vi "input.vi"(8 "error in":errorcluster, 10 "input allocation":T1, 11 "DAQmx Watchdog runtime in":refnum<class "DAQmx Watchdog runtime.lvclass">) -> (0 "error out":errorcluster, 2 "input data":T1, 3 "DAQmx Watchdog runtime out":refnum<class "DAQmx Watchdog runtime.lvclass">)   [LabVIEW 2014, in "DAQmx Watchdog runtime.lvclass"]
doc: "Provides an interface for reading data from a module at runtime. While this interface performs no operations, a child should provide an override which may read from any open sessions, references, or interfaces."
uses:
  DAQmx Watchdog runtime.lvclass
  <vilib>/NI/Tag Bus/table/data table.ctl
  input user data.ctl
  DAQmx Watchdog runtime.lvclass/DAQmx Watchdog runtime.ctl
  <vilib>/NI/Syslog Wrapper - Linux/write syslog.vi
  <vilib>/Utility/LVClass/Get LV Class Name.vi
  <resource>/objmgr/daqmx.rc
  <vilib>/NI/Tag Bus Module Framework/runtime/TBM module execution interface.lvclass
  <vilib>/NI/Tag Bus/table/data table.lvlib
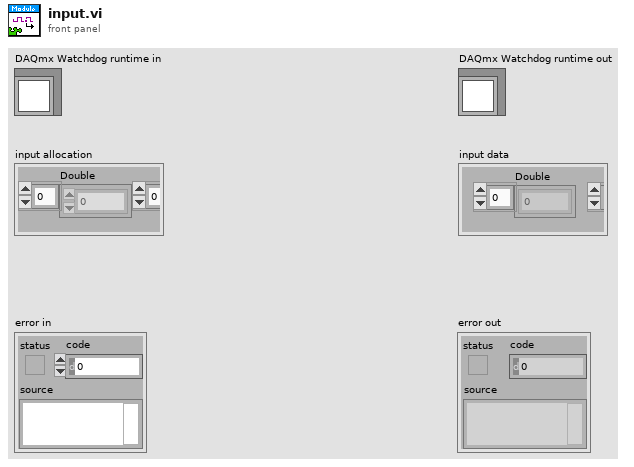
[diagram p1: front panel]
types:
  T1 = typedef "tag bus.lvlib/data table.lvlib/data table.ctl" = cluster{"Double":dbl[], "Single":sgl[], "I64":i64[], "I32":i32[], "I16":i16[], "I8":i8[], "U64":u64[], "U32":u32[], "U16":u16[], "U8":u8[], "Boolean":bool[], "String":string[], "Array of Double":cluster{"DBL Array":dbl[]}[], "Array of Single":cluster{"SGL Array":sgl[]}[], "Array of I64":cluster{"I64 Array":i64[]}[], "Array of I32":cluster{"I32 Array":i32[]}[], "Array of I16":cluster{"I16 Array":i16[]}[], "Array of I8":cluster{"I8 Array":i8[]}[], "Array of U64":cluster{"U64 Array":u64[]}[], "Array of U32":cluster{"U32 Array":u32[]}[], "Array of U16":cluster{"U16 Array":u16[]}[], "Array of U8":cluster{"U8 Array":u8[]}[], "Array of Boolean":cluster{"Boolean Array":bool[]}[], "Array of String":cluster{"String Array":string[]}[]}
  T2 = typedef "DAQmx Watchdog runtime.lvclass/input user data.ctl" = cluster{"Watchdog Expired":bool}
  T3 = typedef "DAQmx Watchdog configuration.lvclass/input data indices.ctl" = cluster{"Boolean.Watchdog Expired":i32}
  T4 = enum16{"Emergency", "Alert", "Critical", "Error", "Warning", "Notice", "Informational", "Debug"}
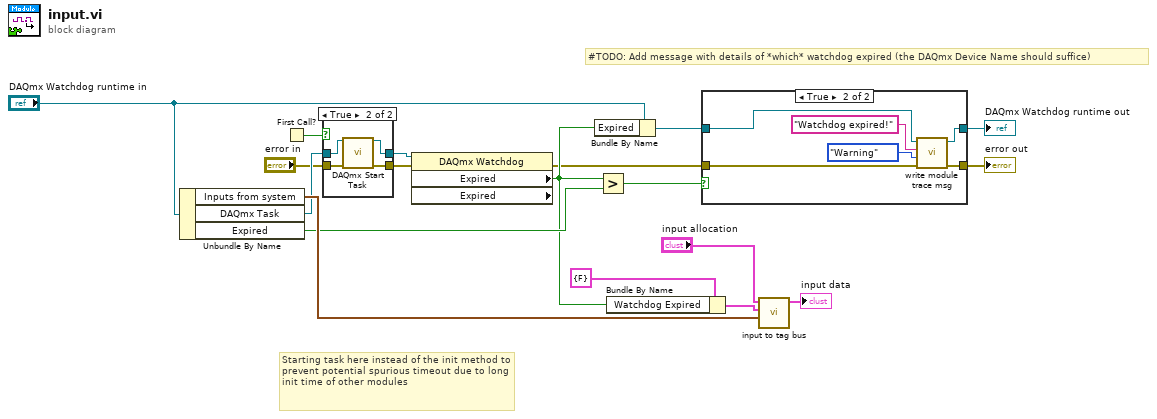
[diagram p0: block diagram]
diagram:
  # "#TODO: Add message with details of *which* watchdog expired (the DAQmx Device Name should suffice)"
  # "Starting task here instead of the init method to prevent potential spurious timeout due to long init time of other modules"
  n1 = Unbundle By Name("DAQmx Watchdog runtime in") -> ("Inputs from system"=w16:T3, "DAQmx Task"=w12:refnum<k21>, "Expired"=w8:bool)
  n2 = First Call?() -> (First Call?: T/F=w13:bool)
  n3 = case shown="True" w13 {
    tunnel: w12 -> [w19 w24]
    tunnel: "error in" -> [w20 w23]
    tunnel: [w20 w22] -> w10
    tunnel: [w19 w21] -> w9
    frame False {
    }
    frame True {
      n4 = call <vilib>:"DAQmx Start Task.vi"("task/channels in"=w24, "error in"=w23) -> ("task out"=w21:refnum<k21>, "error out"=w22:errorcluster)  [unwired: 12 in]
    }
  }
  n5 = property class="DAQmx Watchdog" props=["Expired", "Expired"](reference=w9, error in=w10) -> (error out=w4:errorcluster, "Expired"=w6:bool)  [unwired: 2 out]
  n6 = Bundle By Name(cluster="DAQmx Watchdog runtime in", "Expired"=w6) -> (w5:refnum<class "DAQmx Watchdog runtime.lvclass">)
  n7 = Greater?(x=w6, y=w8) -> (0:w1:bool)
  n8 = Bundle By Name(cluster=T2 {"Watchdog Expired"=FALSE} ("data cluster"), "Watchdog Expired"=w6) -> (w14:T2)
  n9 = case shown="True" w1 {
    tunnel: w5 -> [w25 w32]
    tunnel: w4 -> [w26 w31]
    tunnel: [w26 w30] -> w3
    tunnel: [w25 w27] -> w2
    frame False {
    }
    frame True {
      n10 = call <vilib>:"write module trace msg.vi"("error in (no error)"=w31, "Priority"=T4."Warning", "message"="Watchdog expired!", "module in"=w32) -> ("error out"=w30:errorcluster, "module out"=w27:refnum<class "DAQmx Watchdog runtime.lvclass">)  [unwired: 6 in]
    }
  }
  "error out" <- w3
  "DAQmx Watchdog runtime out" <- w2
  n11 = call "input to tag bus.vi"("indices"=w16, "data cluster"=w14, "tag bus in"="input allocation") -> ("tag bus out"=→"input data":T1)  [unwired: 8 in]
